vi "DynamicLoadNewGraph.vi"(7 "ViewerPath":path, 8 "error in (no error)":errorcluster, 10 "Preferred_tags":string[](array[string]), 11 "Gserver in":refnum<class "Gserver.lvclass">) -> (0 "error out":errorcluster, 3 "Gserver out":refnum<class "Gserver.lvclass">)   [LabVIEW 2020, in "Sgraph_lib_V1.lvlib" / "Gserver.lvclass"]
doc: "Andre Koelewijn, 2 jan 2021\n\nDynamically open a new Gviewer application instance.\nThe name of the new instance depends upon the numbers of open graphs and is determined by Gserver.\nThe maximum number of allowed graphs is defined as provided to this vi."
uses:
  Gserver.lvclass
  Gserver.lvclass/Gserver.ctl
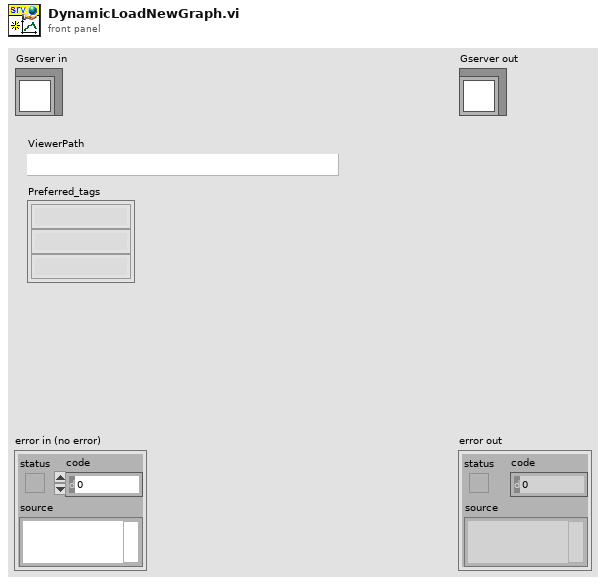
[diagram p1: front panel]
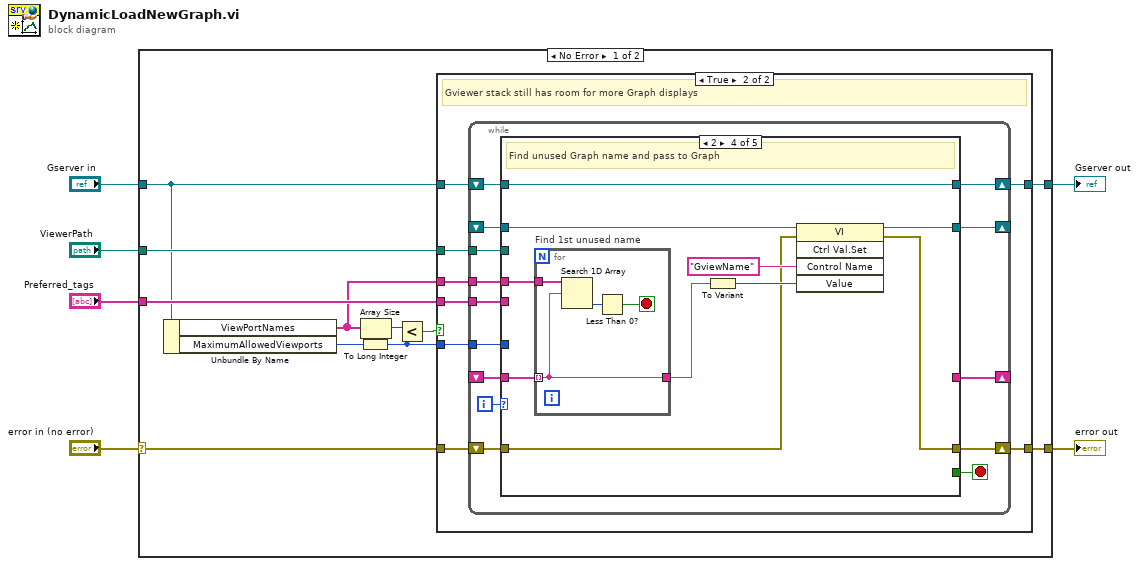
[diagram p0: block diagram]
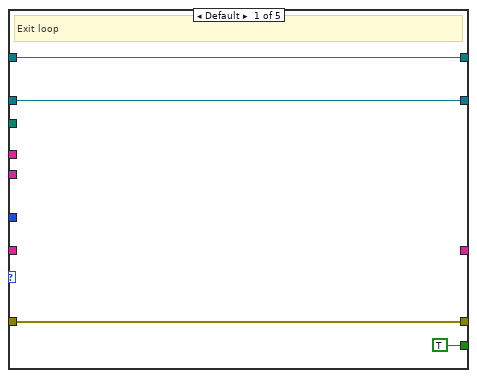
[diagram p3: hidden frame]
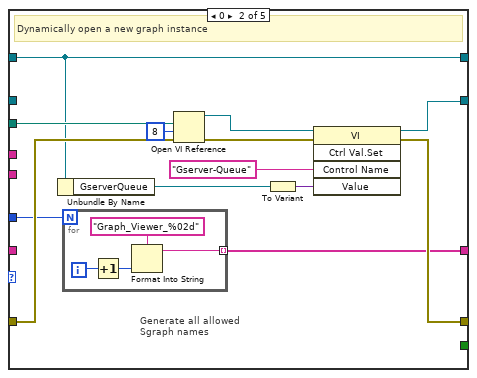
[diagram p4: hidden frame]
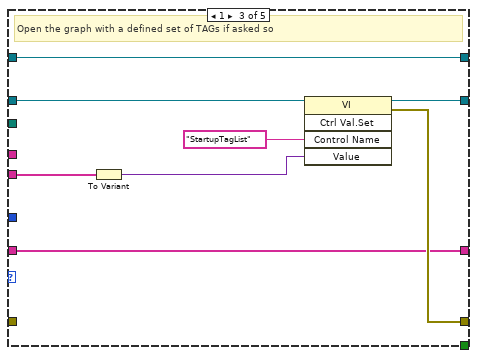
[diagram p5: hidden frame]
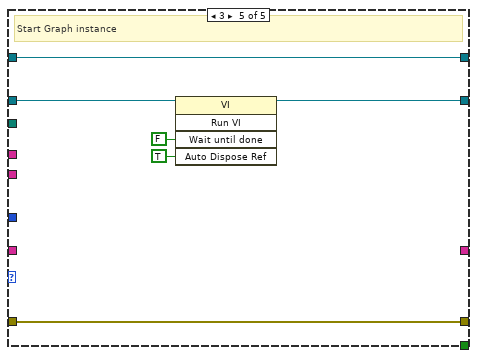
[diagram p6: hidden frame]
diagram:
  n1 = case shown="No Error" "error in (no error)" {
    selector: "error in (no error)" -> [w16 w92]
    tunnel: [w11 w92] -> w5
    tunnel: [w15 w91] -> w3
    tunnel: "Gserver in" -> [w13 w91]
    tunnel: "ViewerPath" -> [w17 _]
    tunnel: "Preferred_tags" -> [w14 _]
    frame No Error {
      n2 = Unbundle By Name(w13) -> ("ViewPortNames"=w7:string[], "MaximumAllowedViewports"=w9:u8)
      n3 = To Long Integer(number=w9) -> (32bit integer=w8:i32)
      n4 = Array Size(array=w7) -> (size(s)=w10:i32)
      n5 = Less?(x=w10, y=w8) -> (x < y?=w12:bool)
      n6 = case shown="True" w12 {
        tunnel: w17 -> [_ w27]
        tunnel: w16 -> [w18 w26]
        tunnel: [w19 w25] -> w15
        tunnel: w14 -> [_ w24]
        tunnel: w13 -> [w19 w23]
        tunnel: [w18 w22] -> w11
        tunnel: w8 -> [_ w21]
        tunnel: w7 -> [_ w20]
        frame False {
          # "Maximum number of Graph displays is reached"
        }
        frame True {
          # "Gviewer stack still has room for more Graph displays"
          n7 = while {
            tunnel: w27 -> [w41]
            shift-right: [w37] -> w25
            shift-left: w23 -> [w38]
            shift-right: [w35] -> w22
            shift-left: w26 -> [w40]
            shift-right: [w36] -> _
            shift-left: _ -> [w34]
            tunnel: w24 -> [w32]
            tunnel: w21 -> [w31]
            shift-right: [w30] -> _
            shift-left: _ -> [w29]
            tunnel: w20 -> [w28]
            i -> [w39]
            stop <- w33 stop-if-true
            n8 = case shown="2" w39 {
              tunnel: w41 -> [_ w58 _ _ _]
              tunnel: w40 -> [w43 w57 _ w74 w89]
              tunnel: w38 -> [w44 w54 w69 w79 w90]
              tunnel: [w44 w54 w69 w79 w90] -> w37
              tunnel: [w45 w49 w66 w76 w85] -> w36
              tunnel: [w43 w50 w67 w77 w89] -> w35
              tunnel: w34 -> [w45 _ w65 w75 w88]
              tunnel: [TRUE _ _ _ _] -> w33
              tunnel: w32 -> [_ _ w64 _ _]
              tunnel: w31 -> [_ w47 _ _ _]
              tunnel: [_ w46 w63 _ _] -> w30
              tunnel: w29 -> [_ _ w63 w72 _]
              tunnel: w28 -> [_ _ _ w73 _]
              frame Default {
                # "Exit loop"
              }
              frame 0 {
                # "Generate all allowed\nSgraph names"
                # "Dynamically open a new graph instance"
                n9 = Unbundle By Name(w54) -> ("GserverQueue"=w53:refnum<queue>)
                n10 = for {
                  N: w47 -> [_]
                  tunnel: [w59] -> w46 mode=indexing
                  i -> [w61]
                  n11 = Increment(x=w61) -> (x+1=w60:i32)
                  n12 = Format Into String(format string="Graph_Viewer_%02d" ("Control Name"), w60) -> (resulting string=w59:string)  [unwired: 2 in, 1 out]
                }
                n13 = Open VI Reference(vi path=w58, options=8, error in (no error)=w57) -> (vi reference=w55:refnum<vi>, error out=w51:errorcluster)  [unwired: 3 in]
                n14 = To Variant(anything=w53) -> (Variant=w52:variant)
                n15 = invoke class="VI" method="Ctrl Val.Set"(reference=w55, error in=w51, "Control Name"="Gserver-Queue", "Value"=w52) -> (reference out=w49:refnum<vi>, error out=w50:errorcluster)  [unwired: 1 in, 3 out]
              }
              frame 1 {
                # "Open the graph with a defined set of TAGs if asked so"
                n16 = To Variant(anything=w64) -> (Variant=w68:variant)
                n17 = invoke class="VI" method="Ctrl Val.Set"(reference=w65, "Control Name"="StartupTagList", "Value"=w68) -> (reference out=w66:refnum<vi>, error out=w67:errorcluster)  [unwired: 2 in, 3 out]
              }
              frame 2 {
                # "Find unused Graph name and pass to Graph"
                n18 = for "Find 1st unused name" {
                  tunnel: w72 -> [w81] mode=indexing
                  tunnel: w73 -> [w82]
                  tunnel: [w81] -> w71
                  stop <- w83 stop-if-true
                  n19 = Search 1D Array(1D array=w82, element=w81) -> (index of element=w84:i32)  [unwired: 1 in]
                  n20 = Less Than 0?(x=w84) -> (x < 0?=w83:bool)
                }
                n21 = To Variant(anything=w71) -> (Variant=w78:variant)
                n22 = invoke class="VI" method="Ctrl Val.Set"(reference=w75, error in=w74, "Control Name"="GviewName", "Value"=w78) -> (reference out=w76:refnum<vi>, error out=w77:errorcluster)  [unwired: 1 in, 3 out]
              }
              frame 3 {
                # "Start Graph instance"
                n23 = invoke class="VI" method="Run VI"(reference=w88, "Wait until done"=FALSE ("Wait Until Done"), "Auto Dispose Ref"=TRUE ("Auto Dispose Reference")) -> (reference out=w85:refnum<vi>)  [unwired: 2 in, 4 out]
              }
            }
          }
        }
      }
    }
    frame Error {
    }
  }
  "error out" <- w5
  "Gserver out" <- w3
